vi "plot all temp channels differential.vi"() -> ()   [LabVIEW 2015]
uses:
  <vilib>/Utility/error.llb/DialogType.ctl
  <vilib>/DAQmx/read.llb/DAQmx Read (Analog 2D DBL NChan NSamp).vi
  <vilib>/Analysis/baseanly.llb/Mean (DBL).vi
  <vilib>/DAQmx/miscellaneous.llb/DAQmx Fill In Error Info.vi
  <vilib>/Utility/file.llb/Write To Spreadsheet File (DBL).vi
  <vilib>/Analysis/NI_AALBase.lvlib
panel:
  out "Waveform Chart 2":T1(graph)
  in  "temp sensor channels":tag="Dev3/ai0:3"
  in  "stop":bool
  in  "error in":errorcluster
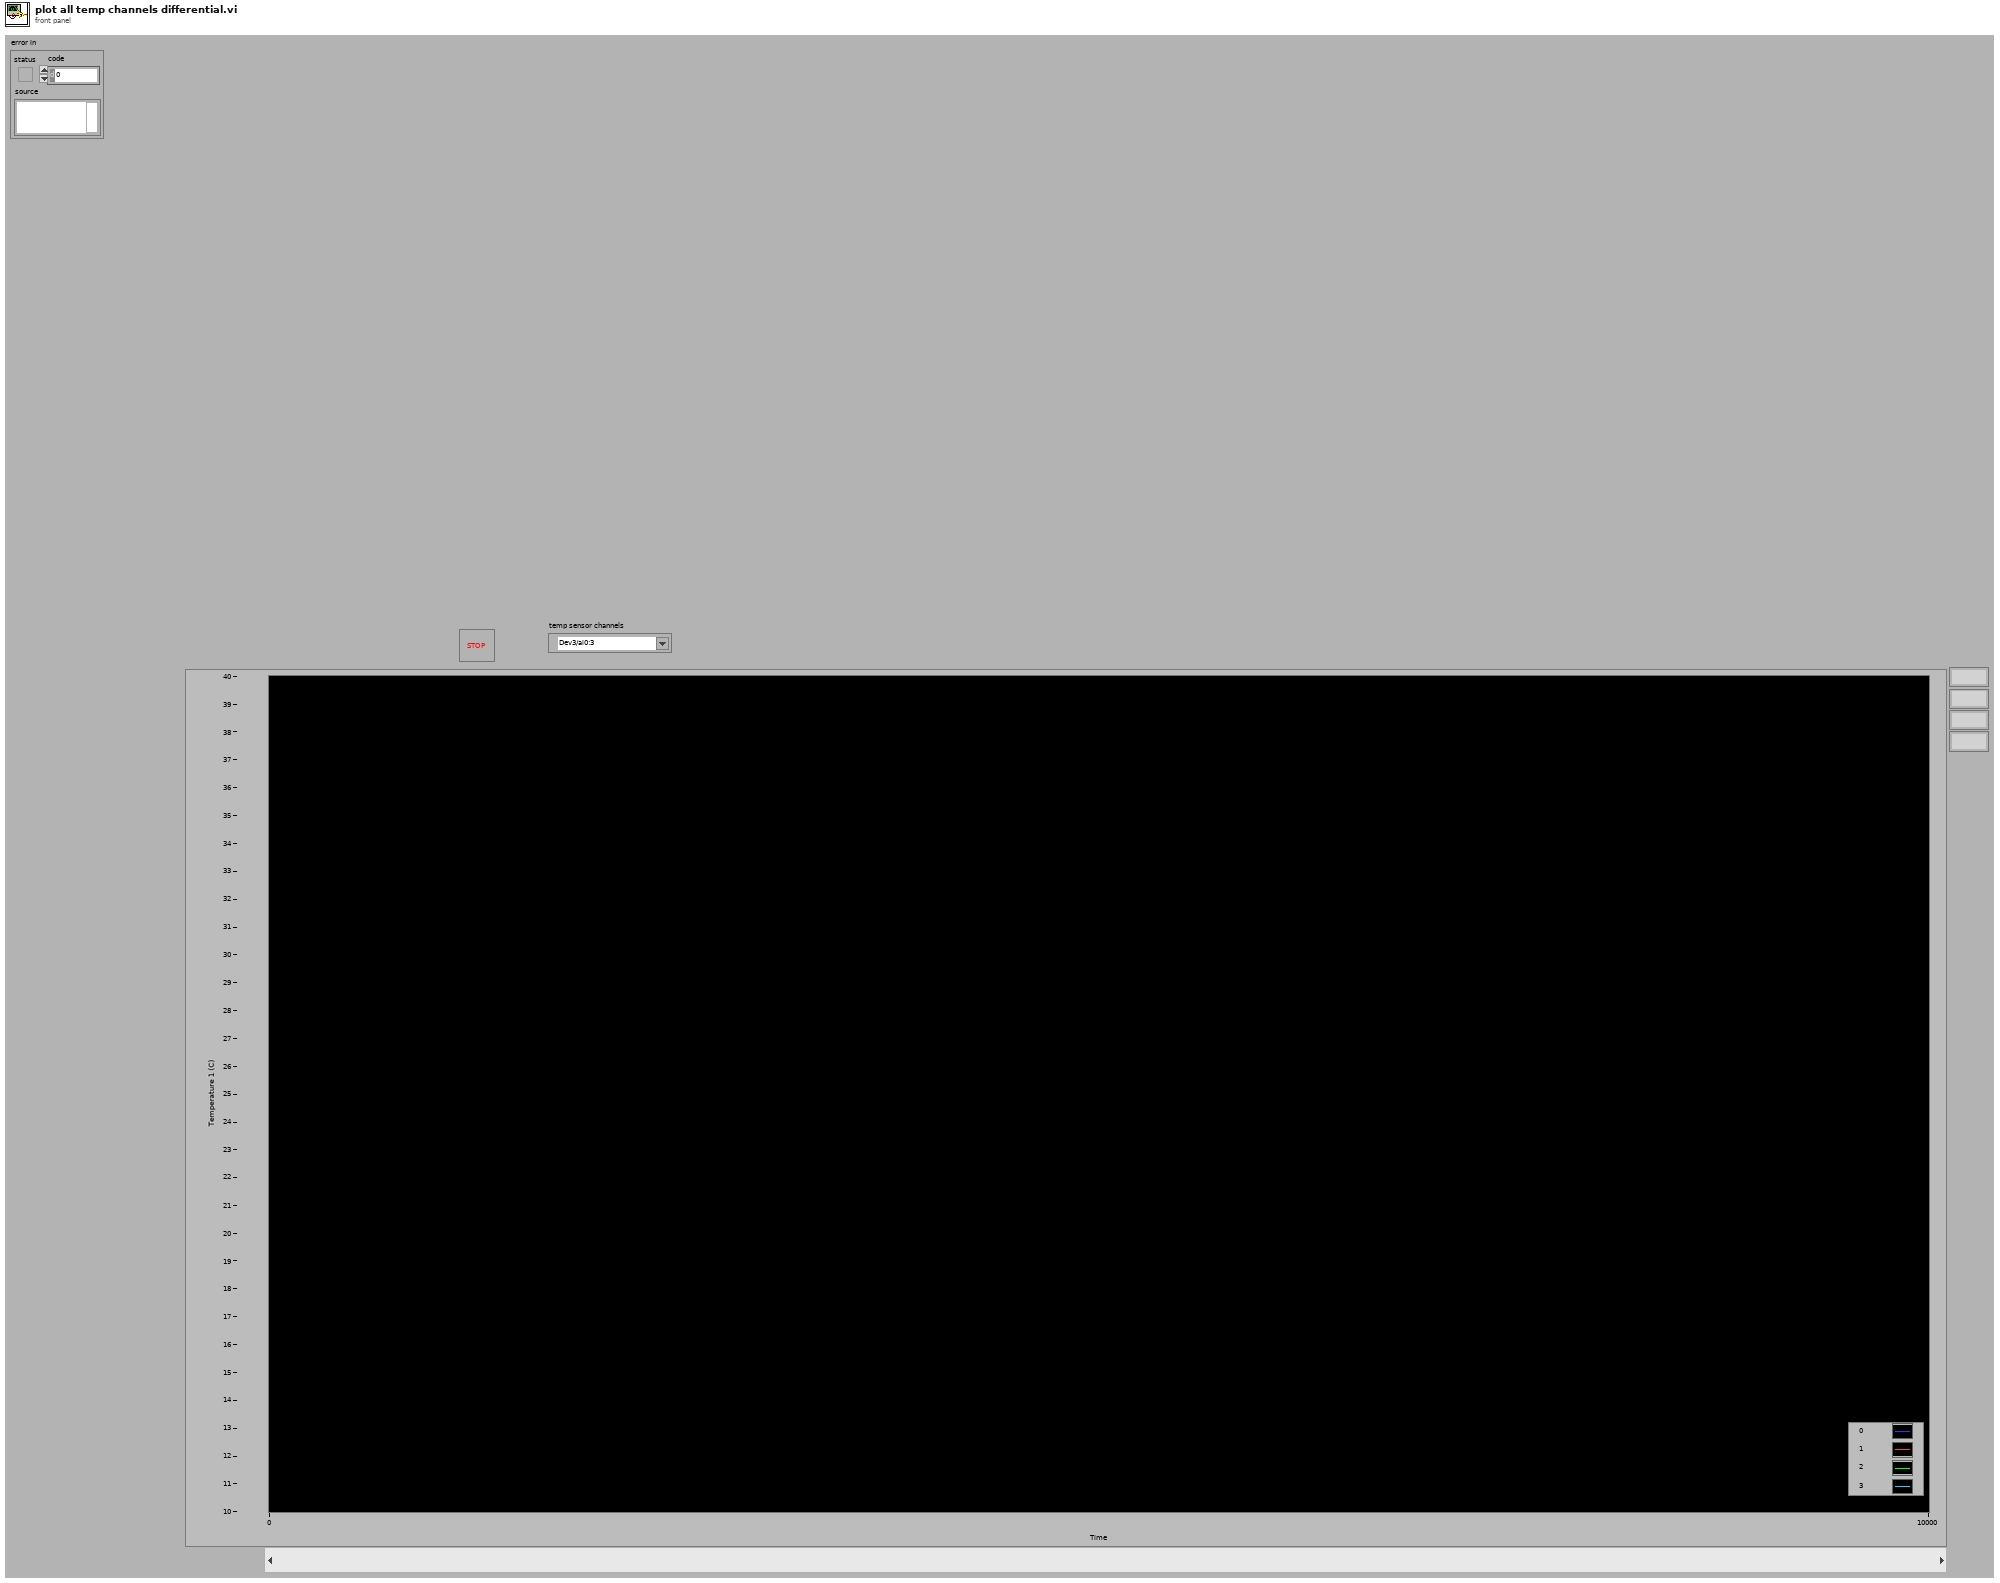
[diagram p1: front panel]
types:
  T1 = cluster{"[0]":dbl, "[1]":dbl, "[2]":dbl, "[3]":dbl}
  T2 = typedef "DialogType.ctl" = u16
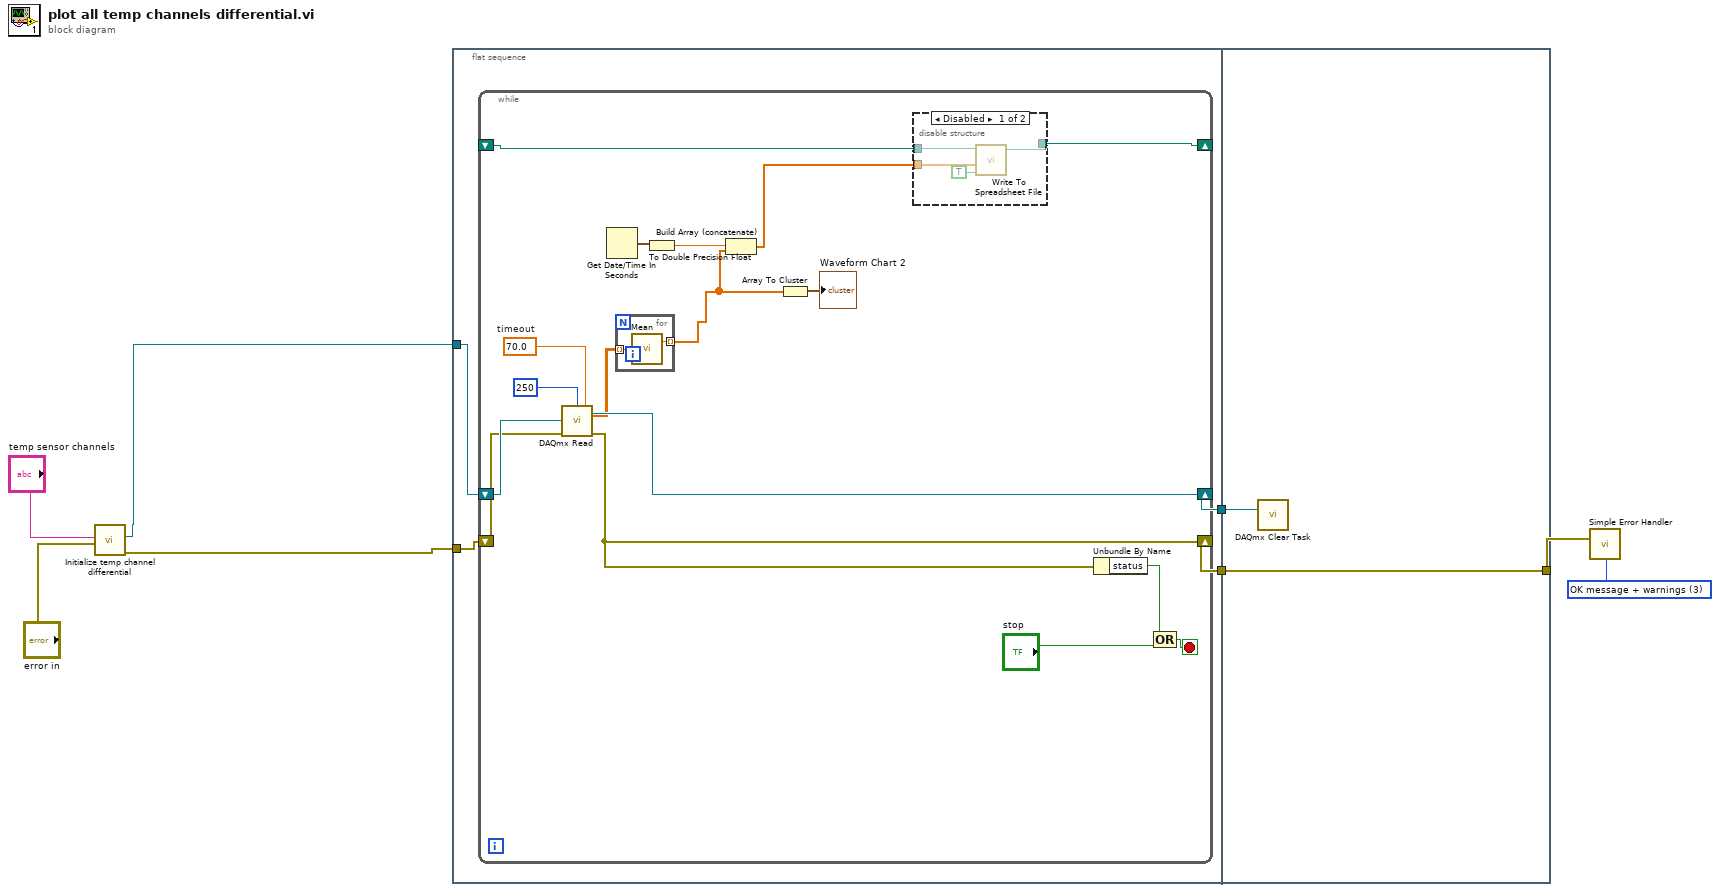
[diagram p0: block diagram]
diagram:
  w7 = T2 3 items=["no dialog", "OK message", "continue or stop message", "OK message + warnings", "continue/stop + warnings"] ("type of dialog (OK msg:1)")
  n1 = call "Initialize temp channel differential.vi"("error in"="error in", "Physical channel"="temp sensor channels") -> ("error out"=w1:errorcluster, "task out"=w2:refnum<k21>)  [unwired: 6 out]
  n2 = flat-sequence {
    tunnel: w2 -> [w12]
    tunnel: [w11] -> w6
    tunnel: [w10] -> w5
    tunnel: w1 -> [w9]
    tunnel: [w37] -> w8
    tunnel: w6 -> [w36]
    tunnel: w5 -> [w37]
    frame #0 {
      n3 = while {
        shift-right: [w13] -> w10
        shift-left: w9 -> [w26]
        shift-right: [w25] -> w11
        shift-left: w12 -> [w27]
        shift-right: [w16] -> _
        shift-left: _ -> [w15]
        stop <- w28 stop-if-true
        w24 = 70.0  # timeout
        n4 = call-poly <vilib>:"DAQmx Read.vi"("task/channels in"=w27, "number of samples per channel"=250, "timeout"=w24, "error in"=w26) -> ("task out"=w25:refnum<k21>, "data"=w22:dbl[][], "error out"=w13:errorcluster)  [unwired: 9 out]
        n5 = Get Date/Time In Seconds() -> (seconds since 1Jan1904=w21:timestamp)
        n6 = for {
          tunnel: [w35] -> w19 mode=indexing
          tunnel: w22 -> [w34] mode=indexing
          n7 = call-poly <vilib>:"Mean.vi"("X"=w34) -> ("mean"=w35:dbl)  [unwired: 1 out]
        }
        n8 = To Double Precision Float(number=w21) -> (double precision float=w18:dbl)
        n9 = Build Array (concatenate)(w18, w19) -> (w14:dbl[])
        n10 = Array To Cluster(array=w19) -> (cluster=→"Waveform Chart 2":T1)
        n11 = disable-structure shown="Disabled" {
          disable-tunnel: [w33 _] -> w16
          disable-tunnel: w15 -> [w32 _]
          disable-tunnel: w14 -> [w31 _]
          frame Disabled {
            n12 = call-poly <vilib>:"Write To Spreadsheet File.vi"("append to file? (new file:F)"=TRUE, "1D data"=w31, "file path (dialog if empty)"=w32) -> ("new file path (Not A Path if cancelled)"=w33:path)  [unwired: 5 in]
          }
          frame Enabled {
          }
        }
        n13 = Unbundle By Name(w13) -> ("status"=w17:bool)
        n14 = Compound Arithmetic op=OR(w17, "stop") -> (w28:bool)
      }
    }
    frame #1 {
      n15 = call <vilib>:"DAQmx Clear Task.vi"("task in"=w36) -> ()  [unwired: 1 in, 14 out]
    }
  }
  n16 = call <vilib>:"Simple Error Handler.vi"("type of dialog (OK msg:1)"=w7, "error in (no error)"=w8) -> ()  [unwired: 8 out]
